vi "_Subsystem_Name Controller.vi"(8 "error in":errorcluster) -> ()   [LabVIEW 2023]
doc: "This VI responds to drive commands both auto and tele Opmodes.\nIt owns the drivebase motors and sensors and runs independent from opModes. Commands can run for arbitrary times, but newly posted commands will interupt as long as Check is called and used for time delays."
uses:
  _Subsystem_Name Operations.ctl
  _Subsystem_Name Setpoints.ctl
  <vilib>/REVLibDriver/REVLibDriver.lvlib
  <resource>/objmgr/REVSpark.rc
  <vilib>/REV Custom Controls/REVSparkRefnum.ctl
  <vilib>/MRC/Types/CmdCtl Completion.ctl
  <vilib>/REV Custom Controls/Spark Output Control Type.ctl
  <vilib>/Rock Robotics/WPI/Framework/Completion Status.ctl
panel:
  in  "Abort Cmd":bool
  in  "Execute Cmd":bool
  in  "Interactive Values":T1
  out "Command Timing":cluster{"Start Time (ms)":u32, "Iterations":i32}
  out "Status":T3
  out "Current Command Data":T1
  out "Cmd Summary":string
  # "Interactive Command: You may fill in the settings for a command\nand schedule it with the Execute button. You can observe and abort\nany command while fine tuning the code for the controller."
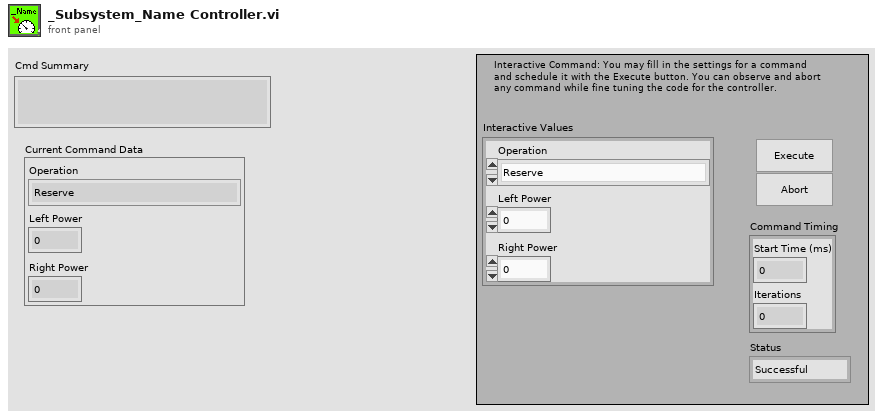
[diagram p1: front panel]
types:
  T1 = typedef "_Subsystem_Name Setpoints.ctl" = cluster{"Operation":T2, "Left Power":dbl, "Right Power":dbl}
  T2 = typedef "_Subsystem_Name Operations.ctl" = enum16{"Reserve", "Read Current", "Immediate"}
  T3 = typedef "Completion Status.ctl" = enum16{"Successful", "Aborted", "Incomplete"}
  T4 = typedef "REVLibDriver.lvlib/REVSparkRefnum.ctl" = refnum<k20>
  T5 = typedef "Command Status Info.ctl" = cluster{"Name":string, "Status":T3, "notifier out":T6}
  T6 = typedef "Completion Notifier.ctl" = refnum<notifier>
  T7 = cluster{"Current Command":T1, "Command Timing":cluster{"Start Time (ms)":u32, "Iterations":i32}, "Command Arguments":cluster{"Command Info":T5, "Description":string, "Default Command":T1, "queue out":refnum<queue>, "Subsystem Name":string}}
  T8 = typedef "REVLibDriver.lvlib/Spark Output Control Type.ctl" = enum16{"Percent VBus", "Velocity", "Voltage", "Position", "Current", "MAXMotion Position", "MAXMotion Velocity"}
  T9 = typedef "CmdCtl Completion.ctl" = enum16{"incomplete", "finished"}
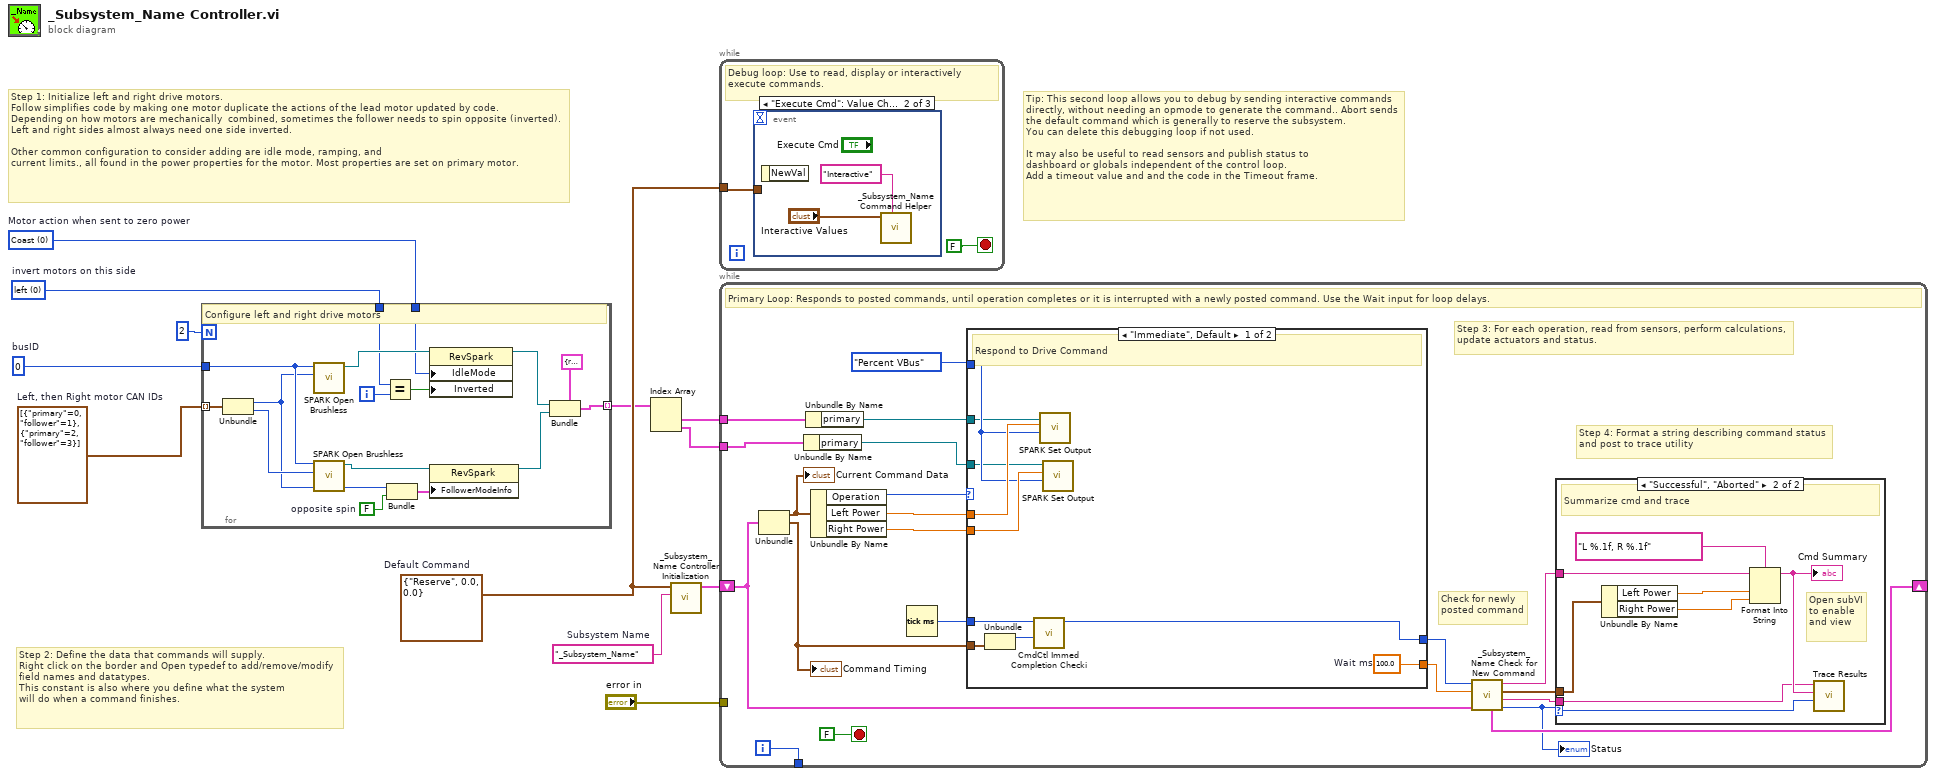
[diagram p0: block diagram]
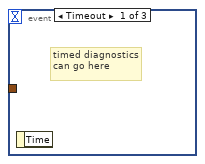
[diagram p2: hidden frame]
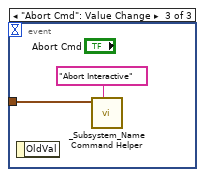
[diagram p3: hidden frame]
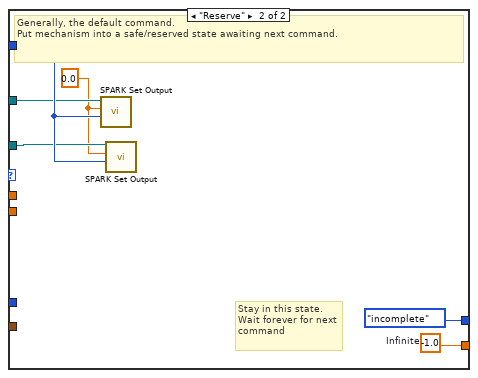
[diagram p5: hidden frame]
diagram:
  w5 = u16 0 items=["left", "right"]  # invert motors on this side
  w6 = cluster{"primary":i32, "follower":i32}[] [{"primary"=0, "follower"=1}, {"primary"=2, "follower"=3}]  # Left, then Right motor CAN IDs
  w7 = 0  # busID
  w9 = u32 0 items=["Coast", "Brake"]  # Motor action when sent to zero power
  w4 = T1 {"Operation"=enum."Reserve", "Left Power"=0.0, "Right Power"=0.0}  # Default Command
  w10 = "_Subsystem_Name"  # Subsystem Name
  # "Tip: This second loop allows you to debug by sending interactive commands\ndirectly, without needing an opmode to generate the command.. Abort sends\nthe default command which is generally to reserve the subsystem.\nYou can delete this debugging loop if not used.\n\nIt may also be useful to read sensors and publish status to\ndashboard or globals independent of the control loop.\nAdd a timeout value and and the code in the Timeout frame."
  # "Step 2: Define the data that commands will supply.\nRight click on the border and Open typedef to add/remove/modify\nfield names and datatypes.\nThis constant is also where you define what the system\nwill do when a command finishes."
  # "Step 1: Initialize left and right drive motors.\nFollow simplifies code by making one motor duplicate the actions of the lead motor updated by code.\nDepending on how motors are mechanically  combined, sometimes the follower needs to spin opposite (inverted).\nLeft and right sides almost always need one side inverted.\n\nOther common configuration to consider adding are idle mode, ramping, and\ncurrent limits., all found in the power properties for the motor. Most properties are set on primary motor."
  n1 = for {
    N: 2 -> [_]
    tunnel: w9 -> [w26]
    tunnel: w7 -> [w25]
    tunnel: w6 -> [w24] mode=indexing
    tunnel: w5 -> [w17]
    tunnel: [w14] -> w3 mode=indexing
    i -> [w19]
    w27 = FALSE  # opposite spin
    # "Configure left and right drive motors"
    n2 = Unbundle(w24) -> ("primary"=w21:i32, "follower"=w23:i32)
    n3 = call <vilib>:"SPARK Open Brushless.vi"("deviceId"=w21, "busID"=w25) -> ("Spark refnum"=w28:T4)  [unwired: 8 in, 1 out]
    n4 = call <vilib>:"SPARK Open Brushless.vi"("deviceId"=w23, "busID"=w25) -> ("Spark refnum"=w22:T4)  [unwired: 8 in, 1 out]
    n5 = Equal?(x=w17, y=w19) -> (x = y?=w18:bool)
    n6 = Bundle("primary"=w21, "opposite spin"=w27) -> (w20:cluster{"primary":i32, "opposite spin ":bool})  [unwired: 1 in]
    n7 = property class="RevSpark"(reference=w28, "IdleMode"=w26, "Inverted"=w18) -> (reference out=w16:T4)  [unwired: 1 in, 1 out]
    n8 = property class="RevSpark"(reference=w22, "FollowerModeInfo"=w20) -> (reference out=w15:T4)  [unwired: 1 in, 1 out]
    n9 = Bundle(cluster=cluster{"primary":T4, "Secondary":T4} {"primary"=refnum, "Secondary"=refnum}, "primary"=w16, "Secondary"=w15) -> (w14:cluster{"primary":T4, "Secondary":T4})
  }
  n10 = Index Array(array=w3) -> (element #1=w2:cluster{"primary":T4, "Secondary":T4}, element #2=w1:cluster{"primary":T4, "Secondary":T4})  [unwired: 2 in]
  n11 = call "_Subsystem_Name Controller Initialization.vi"("Subsystem Name"=w10, "Default Command"=w4) -> ("Current Command"=w11:T7)  [unwired: 9 in]
  n12 = while {
    tunnel: w4 -> [w29]
    stop <- FALSE stop-if-true
    # "Debug loop: Use to read, display or interactively execute commands."
    n13 = event shown="[1] \"Execute Cmd\": Value Change" {
      selector: _ -> [_ _ _]
      dyn-events: _ -> [_ _ _]
      timeout: _ -> [_ _ _]
      tunnel: w29 -> [_ _ w34]
      event Timeout {
        # "timed diagnostics\ncan go here"
        # "Insert Text Here"
        n14 = event-data() -> ()  [unwired: 1 in, 1 out]
      }
      event "Execute Cmd": Value Change {
        # "Execute"
        n15 = event-data() -> ()  [unwired: 1 in, 1 out]
        n16 = call "_Subsystem_Name Command Helper.vi"("Description"="Interactive", "SubSystem Data"="Interactive Values") -> ()  [unwired: 7 in, 3 out]
      }
      event "Abort Cmd": Value Change {
        # "Insert Text Here"
        n17 = event-data() -> ()  [unwired: 1 in, 1 out]
        n18 = call "_Subsystem_Name Command Helper.vi"("Description"="Abort Interactive", "SubSystem Data"=w34) -> ()  [unwired: 7 in, 3 out]
      }
    }
  }
  n19 = while {
    shift-right: [w49] -> _
    shift-left: w11 -> [w43]
    tunnel: [w54] -> _
    tunnel: "error in" -> [_]
    tunnel: w2 -> [w42]
    tunnel: w1 -> [w41]
    i -> [w54]
    stop <- FALSE stop-if-true
    # "Step 4: Format a string describing command status\nand post to trace utility"
    # "Check for newly\nposted command"
    # "Step 3: For each operation, read from sensors, perform calculations,\nupdate actuators and status."
    # "Primary Loop: Responds to posted commands, until operation completes or it is interrupted with a newly posted command. Use the Wait input for loop delays."
    n20 = Unbundle(w43) -> ("Current Command"=w39:T1, "Command Timing"=w40:cluster{"Start Time (ms)":u32, "Iterations":i32})  [unwired: 1 out]
    "Command Timing" <- w40
    "Current Command Data" <- w39
    n21 = Unbundle By Name(w41) -> ("primary"=w35:T4)
    n22 = Unbundle By Name(w42) -> ("primary"=w36:T4)
    n23 = Unbundle By Name(w39) -> ("Operation"=w53:T2, "Left Power"=w52:dbl, "Right Power"=w50:dbl)
    n24 = Tick Count (ms)() -> (millisecond timer value=w51:u32)
    n25 = case shown="\"Immediate\", Default" w53 {
      tunnel: [w73 w79] -> w47
      tunnel: [w70 CmdCtl_Completion."incomplete"] -> w48
      tunnel: w40 -> [w72 _]
      tunnel: w52 -> [w68 _]
      tunnel: w51 -> [w71 _]
      tunnel: w50 -> [w67 _]
      tunnel: Spark_Output_Control_Type."Percent VBus" ("Control Mode") -> [w66 w77]
      tunnel: w36 -> [w65 w76]
      tunnel: w35 -> [w64 w75]
      frame "Immediate", Default {
        w73 = 100.0  # Wait ms
        # "Respond to Drive Command"
        n26 = Unbundle(w72) -> ("Start Time (ms)"=w69:u32)  [unwired: 1 out]
        n27 = call <vilib>:"CmdCtl Immed Completion Checki.vi"("Start Time (ms)"=w69, "current time (ms)"=w71) -> ("Completion"=w70:T9)  [unwired: 9 in]
        n28 = call <vilib>:"SPARK Set Output.vi"("Control Mode"=w66, "Setpoint"=w68, "Spark refnum"=w65) -> ()  [unwired: 7 in, 2 out]
        n29 = call <vilib>:"SPARK Set Output.vi"("Control Mode"=w66, "Setpoint"=w67, "Spark refnum"=w64) -> ()  [unwired: 7 in, 2 out]
      }
      frame "Reserve" {
        w74 = 0.0 ("Setpoint")
        w79 = -1.0  # Infinite
        # "Stay in this state.\nWait forever for next\ncommand"
        # "Generally, the default command.\nPut mechanism into a safe/reserved state awaiting next command."
        n30 = call <vilib>:"SPARK Set Output.vi"("Control Mode"=w77, "Setpoint"=w74, "Spark refnum"=w76) -> ()  [unwired: 7 in, 2 out]
        n31 = call <vilib>:"SPARK Set Output.vi"("Control Mode"=w77, "Setpoint"=w74, "Spark refnum"=w75) -> ()  [unwired: 7 in, 2 out]
      }
    }
    n32 = call "_Subsystem_Name Check for New Command.vi"("Current Command"=w43, "Wait time (ms)"=w47, "Completion"=w48) -> ("Completion"=w38:T3, "Subsystem Name"=w44:string, "Current Command"=w45:T1, "Initial Trace String"=w46:string, "NextCommand"=w49:T7)  [unwired: 4 in]
    "Status" <- w38
    n33 = case shown="\"Successful\", \"Aborted\"" w38 {
      selector: w38 -> [_ w63]
      tunnel: w46 -> [_ w59]
      tunnel: w45 -> [_ w60]
      tunnel: w44 -> [_ w56]
      frame "Incomplete", Default {
        # "Continuing current command"
      }
      frame "Successful", "Aborted" {
        # "Open subVI\nto enable\nand view"
        # "Summarize cmd and trace"
        n34 = Unbundle By Name(w60) -> ("Left Power"=w62:dbl, "Right Power"=w57:dbl)
        n35 = Format Into String(format string="L %.1f, R %.1f", initial string=w59, w62, w57) -> (resulting string=w58:string)  [unwired: 1 in, 1 out]
        "Cmd Summary" <- w58
        n36 = call <vilib>:"Trace Results.vi"("Status of previous command"=w63, "Description"=w58, "Subsystem"=w56) -> ()  [unwired: 9 in]
      }
    }
  }
